vi "Generate Type Definition Filename.vi"(8 "error in":errorcluster, 10 "Name":string, 11 "Path":path) -> (0 "error out":errorcluster, 3 "Typedef Path":path)   [LabVIEW 2026]
doc: "This VI generates a type definition path using the provided typedef name and folder path."
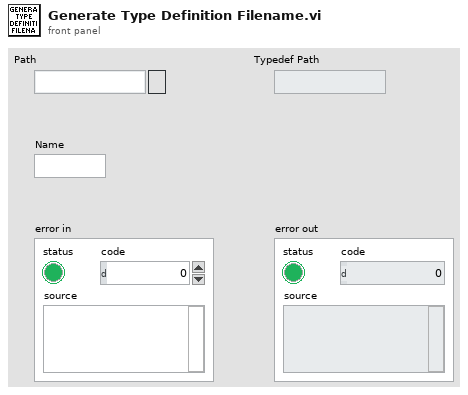
[diagram p1: front panel]
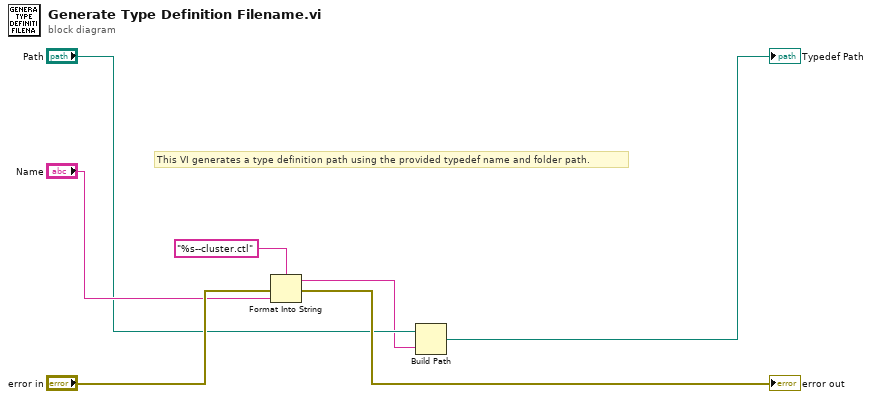
[diagram p0: block diagram]
diagram:
  # "This VI generates a type definition path using the provided typedef name and folder path."
  n1 = Format Into String(format string="%s--cluster.ctl", error in="error in", "Name") -> (resulting string=w2:string, error out=→"error out":errorcluster)  [unwired: 1 in]
  n2 = Build Path(base path="Path", name or relative path=w2) -> (appended path=→"Typedef Path":path)
